vi "test resource not found uri.vi"(8 "error in (no error)":errorcluster) -> (0 "error out":errorcluster, 3 "body":string)   [LabVIEW 2020, in "MCP Server tests.lvlib"]
doc: "A modern resources/read of a uri the server does not have is answered with the JSON-RPC error -32602 whose data is {\"uri\": <the uri asked for>}. The response, like every response of the server, carries the header Connection: close (header name compared case-insensitively). The request is sent with the LabVIEW HTTP Client directly."
uses:
  MCP Server tests.lvlib
  <vilib>/addons/_JKI Toolkits/Caraya/classes/Test/Test.lvclass
  <vilib>/addons/_JKI Toolkits/Caraya/classes/Assert/Assert.lvclass
panel:
  out "lookup error":errorcluster
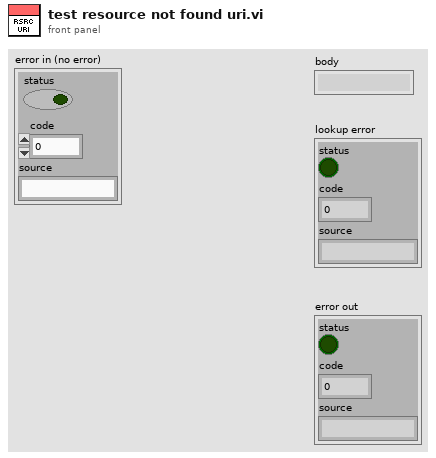
[diagram p1: front panel]
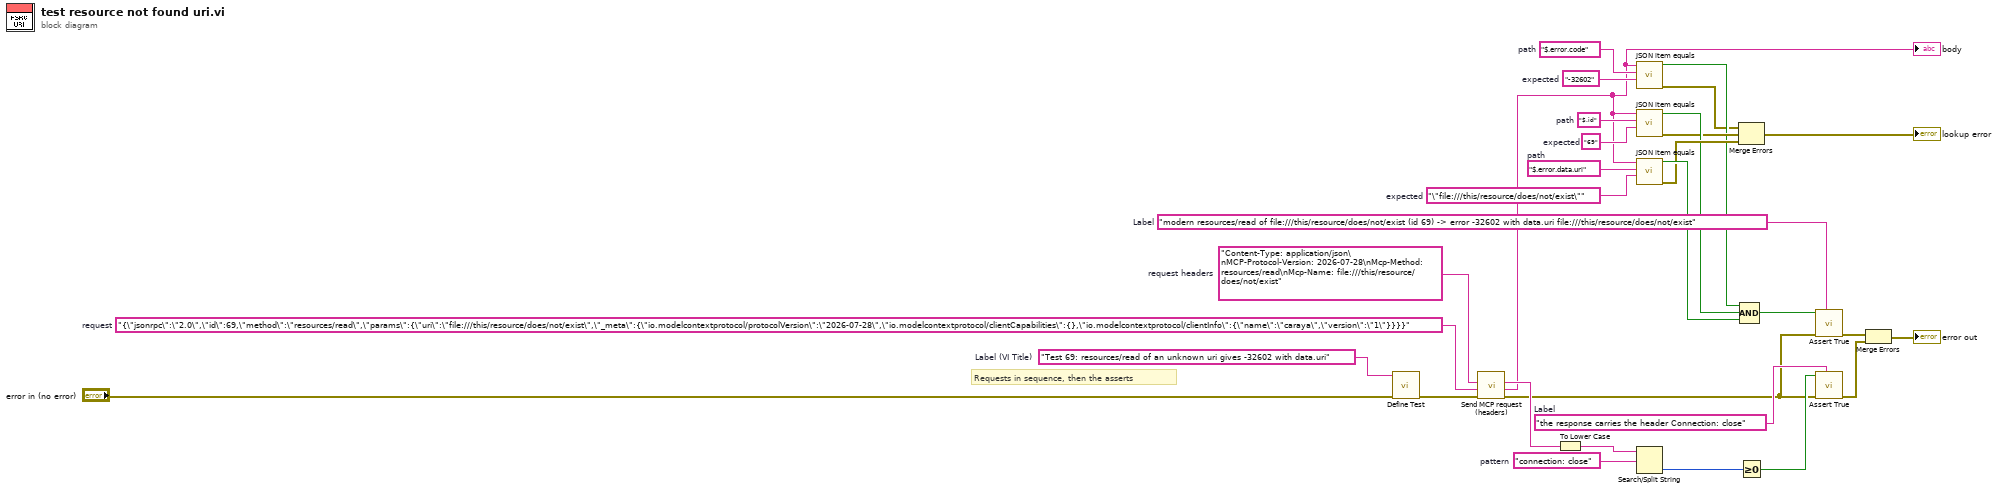
[diagram p0: block diagram]
diagram:
  w29 = "the response carries the header Connection: close"  # Label
  w27 = "modern resources/read of file:///this/resource/does/not/exist (id 69) -> error -32602 with data.uri file:///this/resource/does/not/exist"  # Label
  w22 = "connection: close"  # pattern
  w18 = "\"file:///this/resource/does/not/exist\""  # expected
  w17 = "$.error.data.uri"  # path
  w14 = "69"  # expected
  w13 = "$.id"  # path
  w10 = "-32602"  # expected
  w9 = "$.error.code"  # path
  w5 = "Content-Type: application/json\nMCP-Protocol-Version: 2026-07-28\nMcp-Method: resources/read\nMcp-Name: file:///this/resource/does/not/exist"  # request headers
  w4 = "{\"jsonrpc\":\"2.0\",\"id\":69,\"method\":\"resources/read\",\"params\":{\"uri\":\"file:///this/resource/does/not/exist\",\"_meta\":{\"io.modelcontextprotocol/protocolVersion\":\"2026-07-28\",\"io.modelcontextprotocol/clientCapabilities\":{},\"io.modelcontextprotocol/clientInfo\":{\"name\":\"caraya\",\"version\":\"1\"}}}}"  # request
  w2 = "Test 69: resources/read of an unknown uri gives -32602 with data.uri"  # Label (VI Title)
  # "Requests in sequence, then the asserts"
  n1 = call <vilib>:"Define Test.vi"("error in (no error)"="error in (no error)", "Label (VI Title)"=w2) -> ("error out"=w3:errorcluster)  [unwired: 8 in, 1 out]
  n2 = call "Send MCP request (headers).vi"("error in (no error)"=w3, "request"=w4, "request headers"=w5) -> ("error out"=w6:errorcluster, "response"=w7:string, "headers"=w8:string)  [unwired: 5 in, 1 out]
  "body" <- w7
  n3 = To Lower Case(string=w8) -> (all lower case string=w21:string)
  n4 = call "JSON item equals.vi"("expected"=w10, "path"=w9, "JSON"=w7) -> ("error out"=w11:errorcluster, "equal?"=w12:bool)  [unwired: 6 in, 1 out]
  n5 = call "JSON item equals.vi"("expected"=w14, "path"=w13, "JSON"=w7) -> ("error out"=w15:errorcluster, "equal?"=w16:bool)  [unwired: 6 in, 1 out]
  n6 = call "JSON item equals.vi"("expected"=w18, "path"=w17, "JSON"=w7) -> ("error out"=w19:errorcluster, "equal?"=w20:bool)  [unwired: 6 in, 1 out]
  n7 = Search/Split String(string=w21, search string/char (-)=w22) -> (offset of match=w23:i32)  [unwired: 1 in, 2 out]
  n8 = Merge Errors(w11, w15, w19) -> (→"lookup error":errorcluster)
  n9 = Greater Or Equal To 0?(x=w23) -> (x >= 0?=w24:bool)
  n10 = Compound Arithmetic op=AND(w12, w16, w20) -> (w26:bool)
  n11 = call <vilib>:"Assert True.vi"("Label"=w27, "error in (no error)"=w6, "True?"=w26) -> ("error out"=w28:errorcluster)  [unwired: 7 in, 1 out]
  n12 = call <vilib>:"Assert True.vi"("Label"=w29, "error in (no error)"=w6, "True?"=w24) -> ("error out"=w30:errorcluster)  [unwired: 7 in, 1 out]
  n13 = Merge Errors(w28, w30) -> (→"error out":errorcluster)
